vi "Acqui REG.vi"() -> ()   [LabVIEW 2022 SP3]
uses:
  Variables globales/Variables glob EUROTHERM.vi
  Variables globales/Variable glob generale.vi
panel:
  out "sortie d'erreur":errorcluster
  # "Acqui régulateurs"
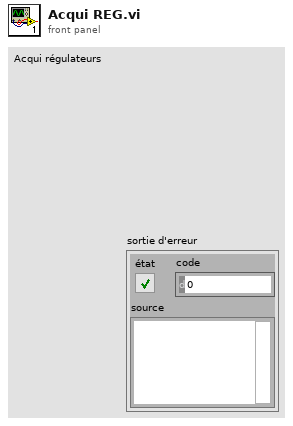
[diagram p1: front panel]
types:
  T1 = typedef "Semaphore RefNum" = refnum<k1>
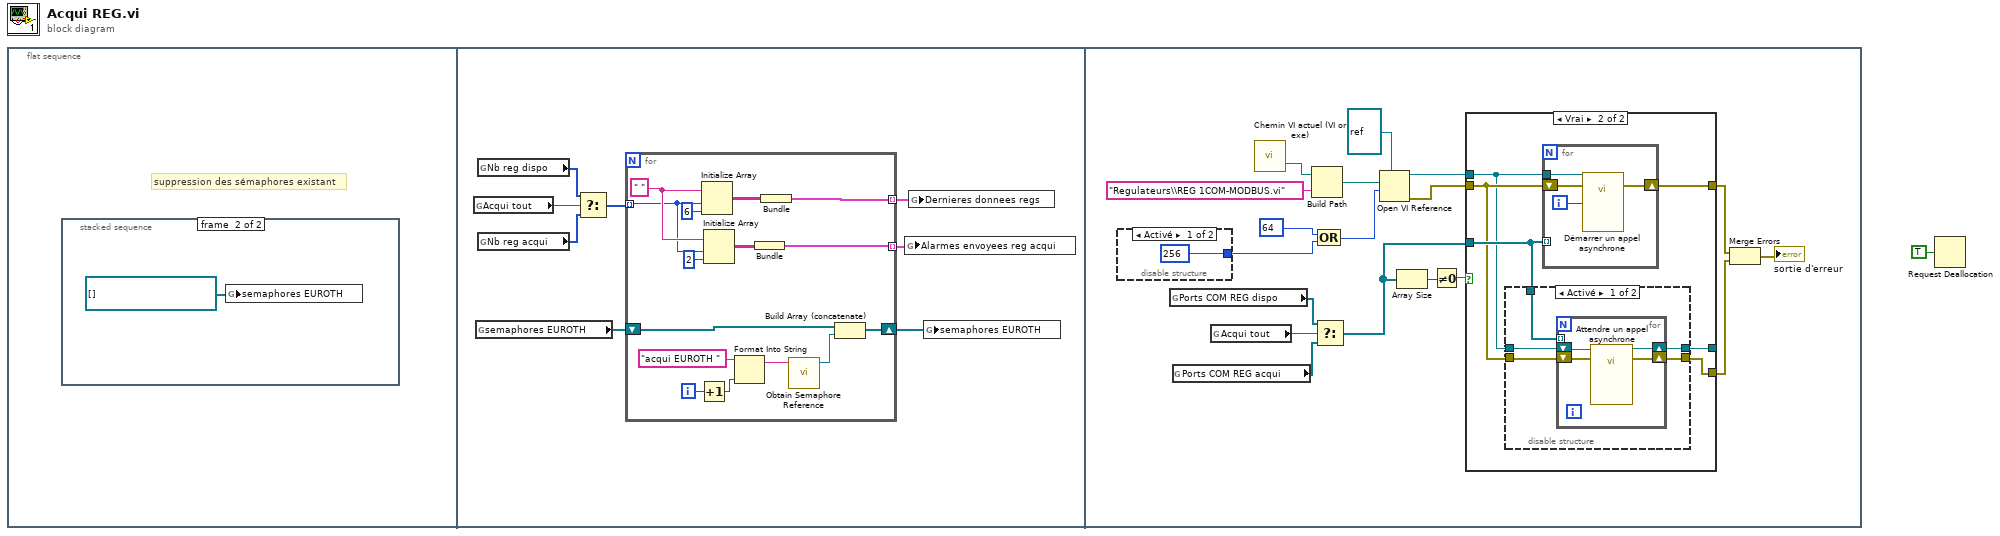
[diagram p0: block diagram]
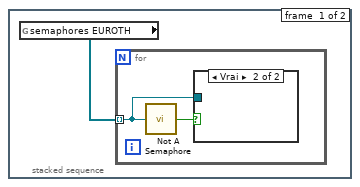
[diagram p2: hidden frame]
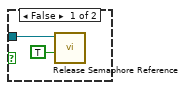
[diagram p3: hidden frame]
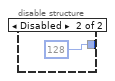
[diagram p4: hidden frame]
diagram:
  n1 = flat-sequence {
    frame #0 {
      # "suppression des sémaphores existant"
      n2 = stacked-sequence {
        frame #0 {
          n3 = global read "Variables glob EUROTHERM.vi" "semaphores EUROTH"() -> (w2:T1[])
          n4 = for {
            tunnel: w2 -> [w3] mode=indexing
            n5 = call <vilib>:"Not A Semaphore.vi"("semaphore"=w3) -> ("not a semaphore"=w4:bool)
            n6 = case shown="Vrai" w4 {
              tunnel: w3 -> [w5 _]
              frame False {
                n7 = call <vilib>:"Release Semaphore Reference.vi"("force destroy? (F)"=TRUE, "semaphore"=w5) -> ()  [unwired: 8 in, 2 out]
              }
              frame True {
              }
            }
          }
        }
        frame #1 {
          w7 = T1[] [] items=["semaphore"] ("semaphores EUROTH")
          n8 = global write "Variables glob EUROTHERM.vi" "semaphores EUROTH"(w7) -> ()
        }
      }
    }
    frame #1 {
      n9 = global read "Variable glob generale.vi" "Acqui tout"() -> (w11:bool)
      n10 = global read "Variables glob EUROTHERM.vi" "semaphores EUROTH"() -> (w15:T1[])
      n11 = global read "Variables glob EUROTHERM.vi" "Nb reg dispo"() -> (w10:u8[])
      n12 = global read "Variables glob EUROTHERM.vi" "Nb reg acqui"() -> (w9:u8[])
      n13 = Select(t=w10, s=w11, f=w9) -> (s? t:f=w8:u8[])
      n14 = for {
        shift-right: [w26] -> w14
        shift-left: w15 -> [w28]
        tunnel: w8 -> [w19] mode=indexing
        tunnel: [w21] -> w13 mode=indexing
        tunnel: [w16] -> w12 mode=indexing
        i -> [w25]
        w20 = " "
        n15 = Increment(x=w25) -> (x+1=w24:i32)
        n16 = Initialize Array(w20, w19, 6 ("taille de la dimension")) -> (w22:string[][])
        n17 = Initialize Array(w20, w19, 2 ("taille de la dimension")) -> (w17:string[][])
        n18 = Format Into String(initial string="acqui EUROTH " ("name (unnamed)"), w24) -> (resulting string=w30:string)  [unwired: 2 in, 1 out]
        n19 = Bundle(w17) -> (w16:cluster{string[][]})  [unwired: 1 in]
        n20 = Bundle(w22) -> (w21:cluster{string[][]})  [unwired: 1 in]
        n21 = call <vilib>:"Obtain Semaphore Reference.vi"("name (unnamed)"=w30) -> ("semaphore"=w27:T1)  [unwired: 4 in, 2 out]
        n22 = Build Array (concatenate)(w28, w27) -> (w26:T1[])
      }
      n23 = global write "Variables glob EUROTHERM.vi" "Alarmes envoyees reg acqui"(w12) -> ()
      n24 = global write "Variables glob EUROTHERM.vi" "Dernieres donnees regs"(w13) -> ()
      n25 = global write "Variables glob EUROTHERM.vi" "semaphores EUROTH"(w14) -> ()
    }
    frame #2 {
      n26 = disable-structure shown="Activé" {
        disable-tunnel: [256 ("options") 128 ("options")] -> w43
        frame Enabled {
        }
        frame Disabled {
        }
      }
      n27 = global read "Variables glob EUROTHERM.vi" "Ports COM REG dispo"() -> (w34:refnum<visa-resource-name>[])
      n28 = global read "Variables glob EUROTHERM.vi" "Ports COM REG acqui"() -> (w33:refnum<visa-resource-name>[])
      n29 = global read "Variable glob generale.vi" "Acqui tout"() -> (w35:bool)
      n30 = call "Chemin VI actuel (VI or exe).vi"() -> ("VI or executable installation directory"=w48:path)  [unwired: 14 in, 1 out]
      n31 = Build Path(base path=w48, name or relative path="Regulateurs\\REG 1COM-MODBUS.vi" ("nom ou chemin relatif")) -> (appended path=w40:path)
      n32 = Select(t=w34, s=w35, f=w33) -> (s? t:f=w32:refnum<visa-resource-name>[])
      n33 = Compound Arithmetic op=OR(64 ("options"), w43) -> (w44:i32)
      n34 = Open VI Reference(type specifier VI Refnum (for type only)=refnum<vi> refnum ("spécificateur de type du refnum de VI (pour type seulement)"), vi path=w40, options=w44) -> (vi reference=w39:refnum<vi>, error out=w45:errorcluster)  [unwired: 3 in]
      n35 = Array Size(array=w32) -> (size(s)=w46:i32)
      n36 = Not Equal To 0?(x=w46) -> (x != 0?=w47:bool)
      n37 = case shown="Vrai" w47 {
        tunnel: w39 -> [w51 w53]
        tunnel: w45 -> [w52 w54]
        tunnel: [w52 w58] -> w38
        tunnel: [w51 w57] -> _
        tunnel: [w52 w56] -> w37
        tunnel: w32 -> [_ w55]
        frame False {
        }
        frame True {
          n38 = disable-structure shown="Activé" {
            disable-tunnel: [w63 w69] -> w57
            disable-tunnel: [w62 w68] -> w56
            disable-tunnel: w55 -> [w61 _]
            disable-tunnel: w54 -> [w60 w68]
            disable-tunnel: w53 -> [w59 w69]
            frame Enabled {
              n39 = for {
                tunnel: w61 -> [_] mode=indexing
                shift-right: [w66] -> w63
                shift-left: w59 -> [w67]
                shift-right: [w64] -> w62
                shift-left: w60 -> [w65]
                n40 = call-by-ref "Attendre un appel asynchrone"(reference=w67, error in=w65) -> (reference out=w66:refnum<vi>, error out=w64:errorcluster)  [unwired: 3 in, 1 out]
              }
            }
            frame Disabled {
            }
          }
          n41 = for {
            tunnel: w55 -> [_] mode=indexing
            shift-right: [w72] -> w58
            shift-left: w54 -> [w73]
            tunnel: w53 -> [w70]
            i -> [w71]
            n42 = call-by-ref "Démarrer un appel asynchrone"(reference=w70, error in=w73, "N° port COM"=w71) -> (error out=w72:errorcluster)  [unwired: 2 in, 2 out]
          }
        }
      }
      n43 = Merge Errors(w38, w37) -> (→"sortie d'erreur":errorcluster)
    }
  }
  n44 = Request Deallocation(TRUE ("flag")) -> ()
